vi "set Y-axis Unit.vi"(8 "error in (no error)":errorcluster, 10 "Y-axis Unit":T1, 11 "FSV-40N in":refnum<class "FSV-40N.lvclass">) -> (0 "error out":errorcluster, 3 "FSV-40N out":refnum<class "FSV-40N.lvclass">)   [LabVIEW 2023, in "Spectrum Analyzer.lvlib" / "FSV-40N.lvclass"]
uses:
  FSV-40N.lvclass
  FSV-40N.lvclass/FSV-40N.ctl
  TYPE DEFINITION/TYPE Y-axis Unit.ctl
  Spectrum Analyzer.lvlib
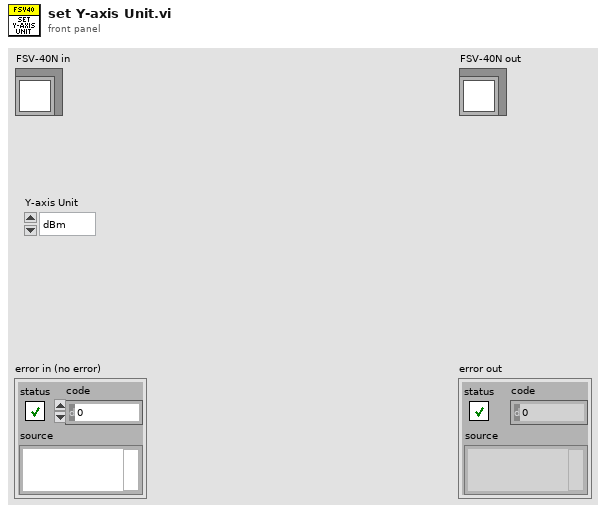
[diagram p1: front panel]
types:
  T1 = typedef "Spectrum Analyzer.lvlib/TYPE Y-axis Unit.ctl" = enum16{"dBm", "dBmV", "dBuV", "dBpW", "Volt", "Ampere", "Watt"}
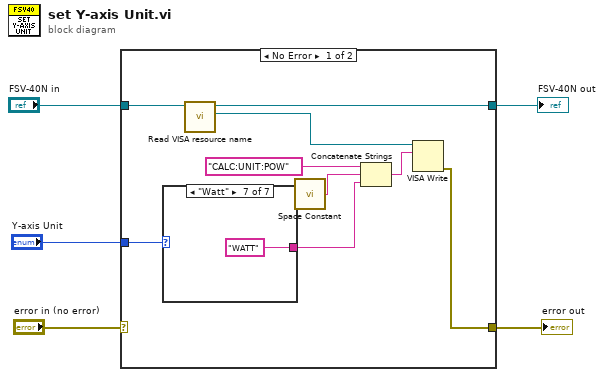
[diagram p0: block diagram]
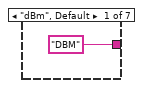
[diagram p2: hidden frame]
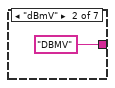
[diagram p3: hidden frame]
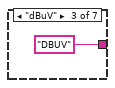
[diagram p4: hidden frame]
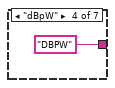
[diagram p5: hidden frame]
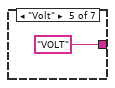
[diagram p6: hidden frame]
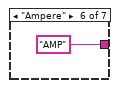
[diagram p7: hidden frame]
diagram:
  n1 = case shown="No Error" "error in (no error)" {
    selector: "error in (no error)" -> [_ w22]
    tunnel: "FSV-40N in" -> [w14 w23]
    tunnel: [w6 w23] -> w3
    tunnel: [w7 w22] -> w2
    tunnel: "Y-axis Unit" -> [w13 _]
    frame No Error {
      n2 = case shown="\"Watt\"" w13 {
        tunnel: ["DBM" "DBMV" "DBUV" "DBPW" "VOLT" "AMP" "WATT"] -> w9
        frame "dBm", Default {
        }
        frame "dBmV" {
        }
        frame "dBuV" {
        }
        frame "dBpW" {
        }
        frame "Volt" {
        }
        frame "Ampere" {
        }
        frame "Watt" {
        }
      }
      n3 = call "Read VISA resource name.vi"("FSV-40N in"=w14) -> ("VISA resource name"=w12:refnum<visa-resource-name>, "FSV-40N out"=w6:refnum<class "FSV-40N.lvclass">)  [unwired: 8 in, 1 out]
      n4 = call <vilib>:"Space Constant.vi"() -> ("String"=w10:string)
      n5 = Concatenate Strings("CALC:UNIT:POW" ("string"), w10, w9) -> (w8:string)
      n6 = VISA Write(VISA resource name=w12, write buffer=w8) -> (error out=w7:errorcluster)  [unwired: 1 in, 2 out]
    }
    frame Error {
    }
  }
  "error out" <- w2
  "FSV-40N out" <- w3
